vi "read data.vi"(11 "Station":string="B_1#FT") -> ()   [LabVIEW 2012]
uses:
  read_Array.vi
panel:
  out "write":u8[](array[numeric])
  out "read":u8[](array[numeric])
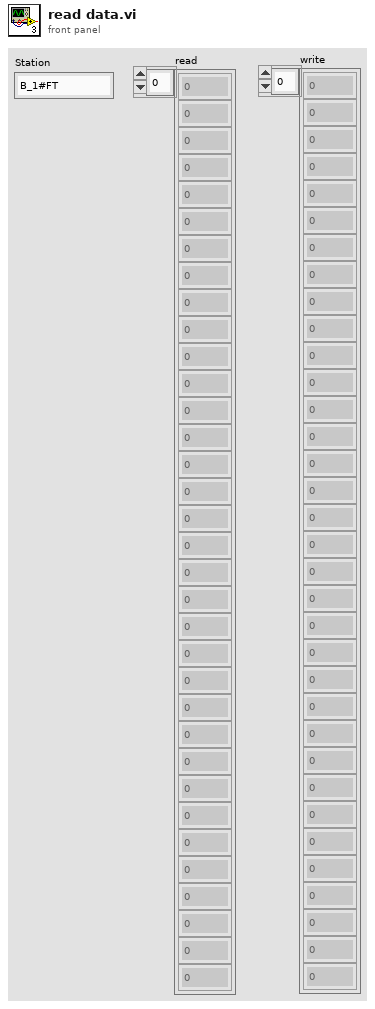
[diagram p1: front panel]
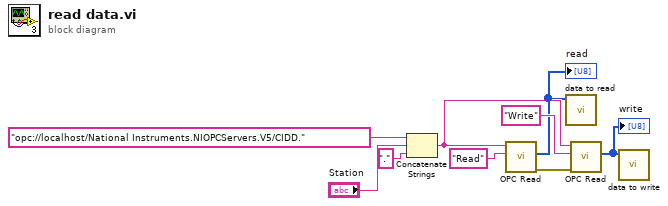
[diagram p0: block diagram]
diagram:
  n1 = Concatenate Strings("opc://localhost/National Instruments.NIOPCServers.V5/CIDD." ("URL"), "Station", "." ("string")) -> (w5:string)
  n2 = call-poly "OPC Read.vi"("Address"="Read", "URL"=w5) -> ("error out"=w3:errorcluster, "Value"=w2:u8[])  [unwired: 7 in, 1 out]
  "read" <- w2
  n3 = call "data to read.vi"("read data"=w2) -> ()  [unwired: 8 in, 3 out]
  n4 = call-poly "OPC Read.vi"("错误输入（无错误）"=w3, "Address"="Write", "URL"=w5) -> ("Value"=w1:u8[])  [unwired: 6 in, 2 out]
  "write" <- w1
  n5 = call "data to write.vi"("write data"=w1) -> ()  [unwired: 11 in]
